vi "WaitOnTestComplete.vi"(8 "error in (no error)":errorcluster, 11 "TestSuite in":refnum<class "TestSuite.lvclass">) -> (0 "error out":errorcluster, 3 "TestSuite out":refnum<class "TestSuite.lvclass">)   [LabVIEW 2013, in "TestSuite.lvclass"]
doc: "Insert WaitOnTestComplete at the end of setUp test hook if the test hook VI opens any references that are needed by the test methods at run time."
uses:
  TestSuite.lvclass
  TestSuite.lvclass/TestSuite.ctl
panel:
  # "JKI VI Tester for LabVIEW\nhttp://jkisoft.com/vi-tester\nCopyright (C) 2007-2009, JKI <info@jkisoft.com>\nALL RIGHTS RESERVED"
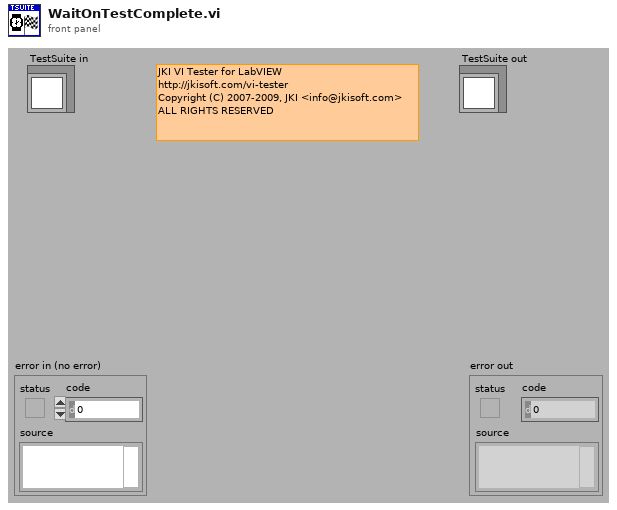
[diagram p1: front panel]
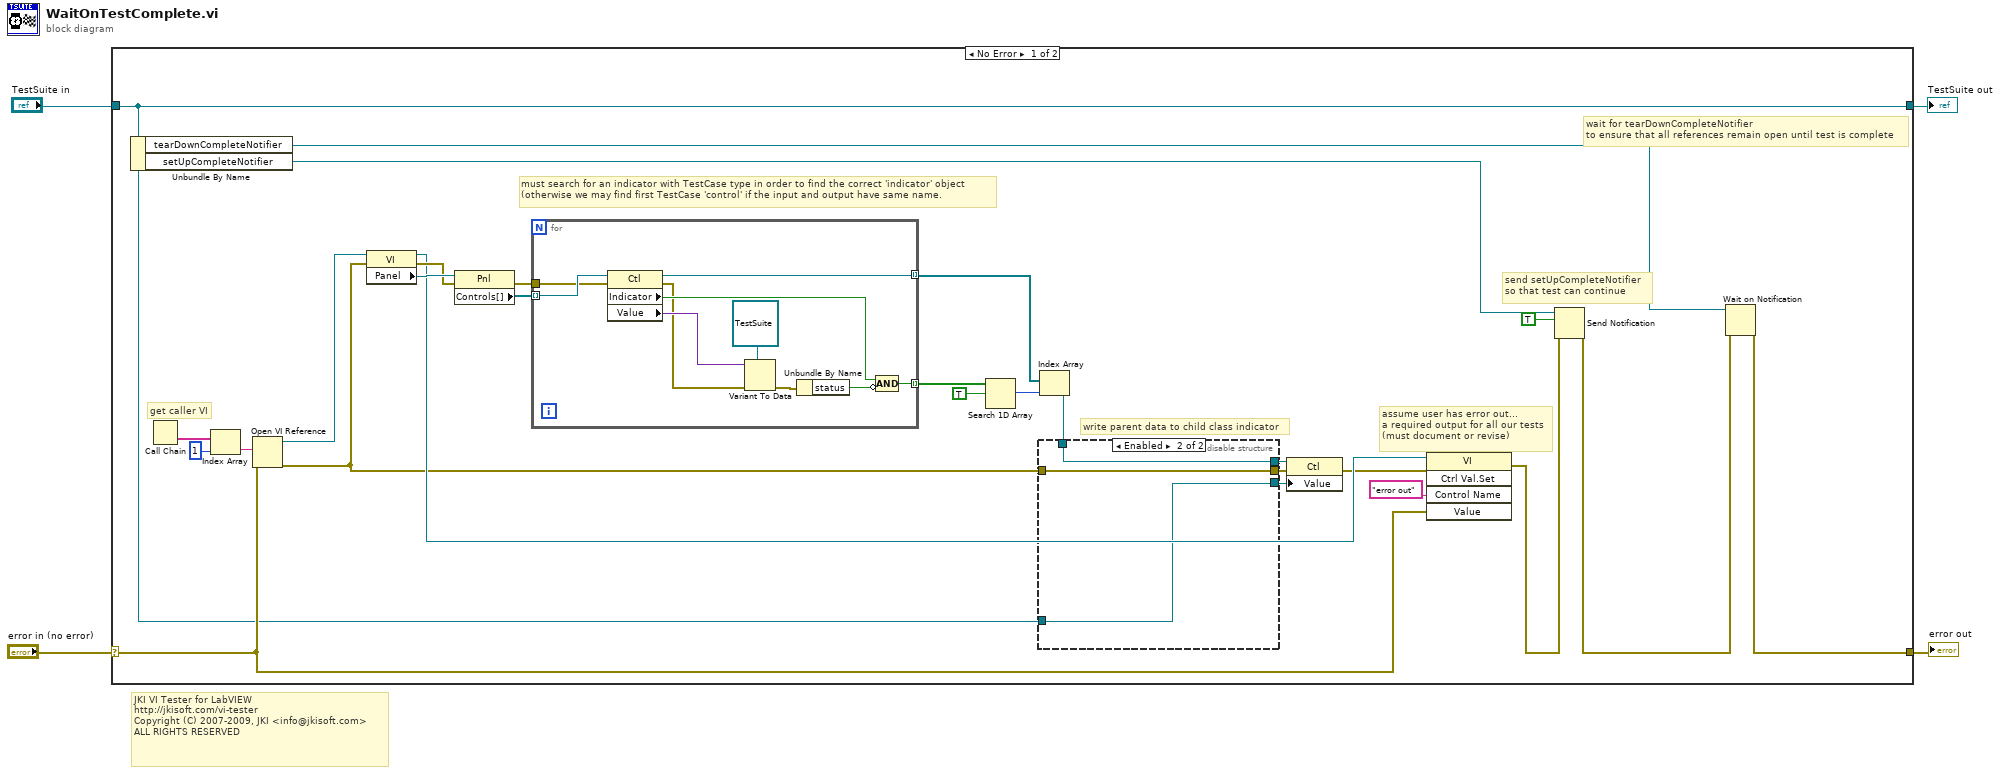
[diagram p0: block diagram]
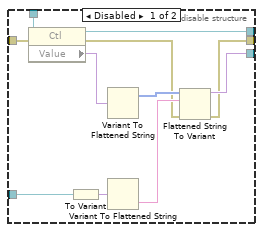
[diagram p2: hidden frame]
diagram:
  # "JKI VI Tester for LabVIEW\nhttp://jkisoft.com/vi-tester\nCopyright (C) 2007-2009, JKI <info@jkisoft.com>\nALL RIGHTS RESERVED"
  n1 = case shown="No Error" "error in (no error)" {
    selector: "error in (no error)" -> [w13 w58]
    tunnel: [w31 w58] -> w3
    tunnel: [w7 w57] -> w1
    tunnel: "TestSuite in" -> [w7 w57]
    frame No Error {
      # "write parent data to child class indicator"
      # "get caller VI"
      # "must search for an indicator with TestCase type in order to find the correct 'indicator' object\n(otherwise we may find first TestCase 'control' if the input and output have same name."
      # "assume user has error out...\na required output for all our tests\n(must document or revise)"
      # "wait for tearDownCompleteNotifier\nto ensure that all references remain open until test is complete"
      # "send setUpCompleteNotifier\nso that test can continue"
      n2 = Unbundle By Name(w7) -> ("tearDownCompleteNotifier"=w32:refnum<notifier>, "setUpCompleteNotifier"=w30:refnum<notifier>)
      n3 = Call Chain() -> (call chain=w27:string[])
      n4 = Index Array(array=w27, index=1) -> (element=w25:string)
      n5 = Open VI Reference(vi path=w25, error in (no error)=w13) -> (vi reference=w12:refnum<vi>, error out=w8:errorcluster)  [unwired: 4 in]
      n6 = property class="VI"(reference=w12, error in=w8) -> (reference out=w15:refnum<vi>, error out=w22:errorcluster, "Panel"=w24:refnum<vi>)
      n7 = property class="Pnl"(reference=w24, error in=w22) -> (error out=w21:errorcluster, "Controls[]"=w23:refnum<vi>[])  [unwired: 1 out]
      n8 = for {
        tunnel: w23 -> [w56] mode=indexing
        tunnel: [w51] -> w20 mode=indexing
        tunnel: w21 -> [w49]
        tunnel: [w48] -> w17 mode=indexing
        n9 = property class="Ctl"(reference=w56, error in=w49) -> (reference out=w48:refnum<vi>, error out=w50:errorcluster, "Indicator"=w52:bool, "Value"=w55:variant)
        n10 = Variant To Data(error in=w50, type=refnum<class "TestSuite.lvclass"> refnum ("reference in"), Variant=w55) -> (error out=w54:errorcluster)  [unwired: 1 out]
        n11 = Unbundle By Name(w54) -> ("status"=w53:bool)
        n12 = Compound Arithmetic op=AND(w52, invert w53) -> (w51:bool)
      }
      n13 = Search 1D Array(1D array=w20, element=TRUE) -> (index of element=w18:i32)  [unwired: 1 in]
      n14 = Index Array(array=w17, index=w18) -> (element=w5:refnum<vi>)
      n15 = disable-structure shown="Enabled" {
        disable-tunnel: [w40 w45] -> w11
        disable-tunnel: [w39 w44] -> w10
        disable-tunnel: [w36 w46] -> w9
        disable-tunnel: w8 -> [w35 w46]
        disable-tunnel: w7 -> [w34 w44]
        disable-tunnel: w5 -> [w33 w45]
        frame Disabled {
          n16 = property class="Ctl"(reference=w33, error in=w35) -> (reference out=w40:refnum<vi>, error out=w37:errorcluster, "Value"=w43:variant)
          n17 = To Variant(anything=w34) -> (Variant=w38:variant)
          n18 = Variant To Flattened String(Variant=w43) -> (1:w42:i16[])  [unwired: 1 out]
          n19 = Variant To Flattened String(Variant=w38) -> (data string=w41:string)  [unwired: 1 out]
          n20 = Flattened String To Variant(4:w37, 6:w41, 7:w42) -> (0:w36:errorcluster, 3:w39:variant)
        }
        frame Enabled {
        }
      }
      n21 = property class="Ctl"(reference=w11, error in=w9, "Value"=w10) -> (error out=w6:errorcluster)  [unwired: 1 out]
      n22 = invoke class="VI" method="Ctrl Val.Set"(reference=w15, error in=w6, "Control Name"="error out", "Value"=w13) -> (error out=w14:errorcluster)  [unwired: 1 in, 4 out]
      n23 = Send Notification(notification=TRUE, notifier=w30, error in (no error)=w14) -> (error out=w29:errorcluster)  [unwired: 1 out]
      n24 = Wait on Notification(notifier=w32, error in (no error)=w29) -> (error out=w31:errorcluster)  [unwired: 2 in, 3 out]
    }
    frame Error {
    }
  }
  "error out" <- w3
  "TestSuite out" <- w1
